vi "xnet_canopen_get_last_error.vi"(8 "error in (no error)":errorcluster, 11 "xnet_co_handle_in":u64) -> (0 "error out":errorcluster, 3 "xnet_co_handle":u64)   [LabVIEW 2023, in "xnet_canopen.lvlib"]
uses:
  xnet_canopen.lvlib
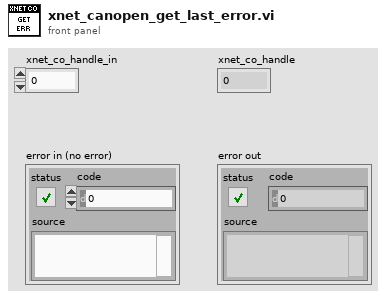
[diagram p1: front panel]
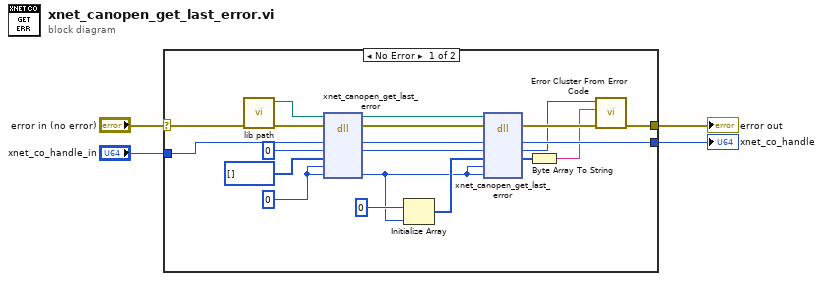
[diagram p0: block diagram]
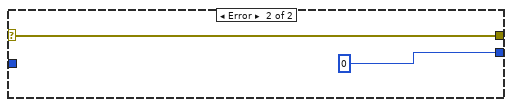
[diagram p2: hidden frame]
diagram:
  n1 = case shown="No Error" "error in (no error)" {
    selector: "error in (no error)" -> [w21 w25]
    tunnel: [w7 w25] -> w3
    tunnel: [w9 u64 0 ("phandle")] -> w2
    tunnel: "xnet_co_handle_in" -> [w22 _]
    frame No Error {
      w18 = u32 0 ("bufsize")
      n2 = call "lib path.vi"() -> ("lib path"=w23:path)  [unwired: 11 in]
      n3 = dll-call lib="?" fn="xnet_canopen_get_last_error"(path in=w23, error in=w21, "handle"=w22, "err_code"=0, "msg"=u8[] [] ("buffer"), "msg_sz"=w18, "expect_size"=w18) -> (path out=w14:path, error out=w16:errorcluster, "handle"=w10:u64, "err_code"=w11:i32, "expect_size"=w12:u32)  [unwired: 4 in]
      n4 = Initialize Array(u8 0 ("element"), w12) -> (w13:u8[])
      n5 = dll-call lib="?" fn="xnet_canopen_get_last_error"(path in=w14, error in=w16, "handle"=w10, "err_code"=w11, "msg"=w13, "msg_sz"=w12, "expect_size"=w12) -> (error out=w15:errorcluster, "handle"=w9:u64, "err_code"=w6:i32, "msg"=w8:u8[])  [unwired: 4 in, 1 out]
      n6 = Byte Array To String(unsigned byte array=w8) -> (string=w5:string)
      n7 = call <vilib>:"Error Cluster From Error Code.vi"("error in (no error)"=w15, "error message (\"\")"=w5, "error code (0)"=w6) -> ("error out"=w7:errorcluster)  [unwired: 6 in]
    }
    frame Error {
    }
  }
  "error out" <- w3
  "xnet_co_handle" <- w2
